vi "flush point buffer to channel.vi"(10 "point buffer":refnum<data-value>, 11 "channel":refnum<class "Channel.lvclass">) -> (0 "error out":errorcluster)   [LabVIEW 2020, in "nominal core steps.lvlib"]
doc: "Streams the content of the point buffer to the specified channel.\nDoes not free data if an error occurs."
uses:
  nominal core steps.lvlib
  <vilib>/Nominal/Nominal IO Client/submodules/nominal-streaming-labview-ffi/lv_src/Channel/Channel.lvclass
  points buffer.ctl
  single point.ctl
  <vilib>/Nominal/Nominal IO Client/submodules/nominal-streaming-labview-ffi/lv_src/Channel/Push Points Batch_XY.vi
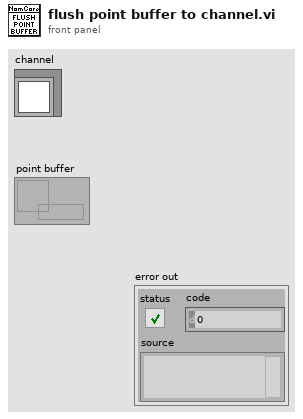
[diagram p1: front panel]
types:
  T1 = typedef "nominal core steps.lvlib/points buffer.ctl" = T2[]
  T2 = typedef "nominal core steps.lvlib/single point.ctl" = cluster{"Time Stamp":timestamp, "Value":dbl}
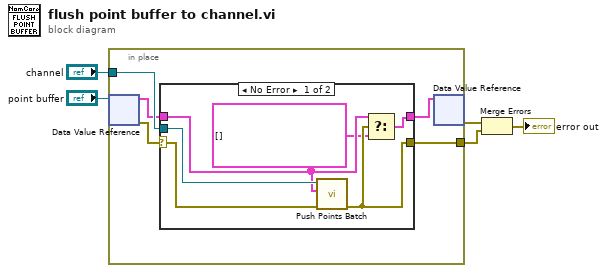
[diagram p0: block diagram]
diagram:
  n1 = in-place {
    in-place-border: "channel" -> [w10]
    in-place-border: [w6] -> w2
    n2 = in-place-dvr #1("point buffer") -> (w7:T1, w9:errorcluster)
    n3 = case shown="No Error" w9 {
      selector: w9 -> [w15 w17]
      tunnel: w10 -> [w16 _]
      tunnel: [w11 w18] -> w8
      tunnel: w7 -> [w13 w18]
      tunnel: [w14 w17] -> w6
      frame No Error {
        n4 = call-poly <vilib>:"Push Points Batch.vi"("error in (no error)"=w15, "Points"=w13, "Channel in"=w16) -> ("error out"=w14:errorcluster)  [unwired: 7 in, 1 out]
        n5 = Select(t=w13, s=w14, f=cluster{"Time Stamp":timestamp, "Value":dbl}[] []) -> (s? t:f=w11:T1)
      }
      frame Error {
      }
    }
    n6 = in-place-dvr #1(w8) -> (w3:errorcluster)  [unwired: 1 out]
  }
  n7 = Merge Errors(w3, w2) -> (→"error out":errorcluster)
